vi "OwnCompat20261012_Native_GetCaseFrameNames.vi"() -> ()   [LabVIEW 2024]
panel:
  out "error out":errorcluster caption="错误输出"
  out "frame_names":string[](array[string])
  in  "case_id":u32
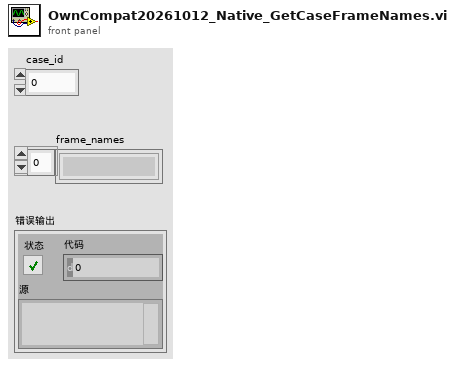
[diagram p1: front panel]
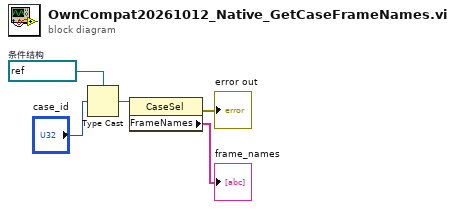
[diagram p0: block diagram]
diagram:
  w4 = refnum<vi> refnum  # 条件结构
  n1 = Type Cast ("强制类型转换")(type=w4, x="case_id") -> (*(type *) &x=w3:refnum<vi>)
  n2 = property on="属性节点" class="CaseSel"(reference=w3) -> (error out=→"error out":errorcluster, "FrameNames"=→"frame_names":string[])  [unwired: 1 in, 1 out]
